vi "Ch_Apply.vi"(0 "Channels":T1(array[cluster]), 5 "Index":i32, 7 "Channel":T2={"Name"="CH000", "Value"=0.0, "High Limit"=100.0, "Low Limit"=0.0, "Save"=TRUE, "Graph"=FALSE, "Scale Min"=0.0, "Scale Max"=100.0, "Unit"="%"}, 9 "Apply All":bool, 11 "error in":errorcluster) -> (4 "Channels out":T1(array[cluster]), 15 "error out":errorcluster)   [LabVIEW 2026]
doc: "채널 설정 팝업 결과 반영: Apply All이면 상/하한·저장·그래프·스케일·단위를 128채널 모두에(이름/값 유지), 아니면 Index 채널만 교체."
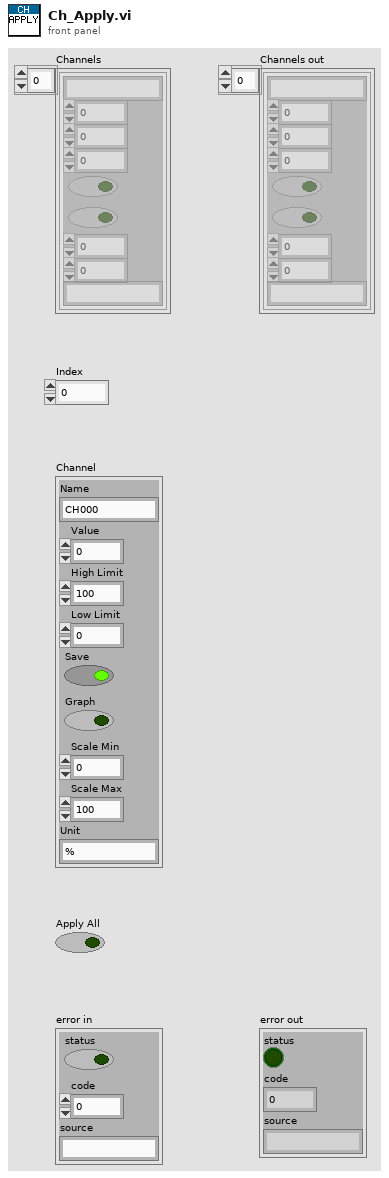
[diagram p1: front panel]
types:
  T1 = cluster{"Name":string, "Value":dbl, "High Limit":dbl, "Low Limit":dbl, "Save":bool, "Graph":bool, "Scale Min":dbl, "Scale Max":dbl, "Unit":string}[]
  T2 = cluster{"Name":string, "Value":dbl, "High Limit":dbl, "Low Limit":dbl, "Save":bool, "Graph":bool, "Scale Min":dbl, "Scale Max":dbl, "Unit":string}
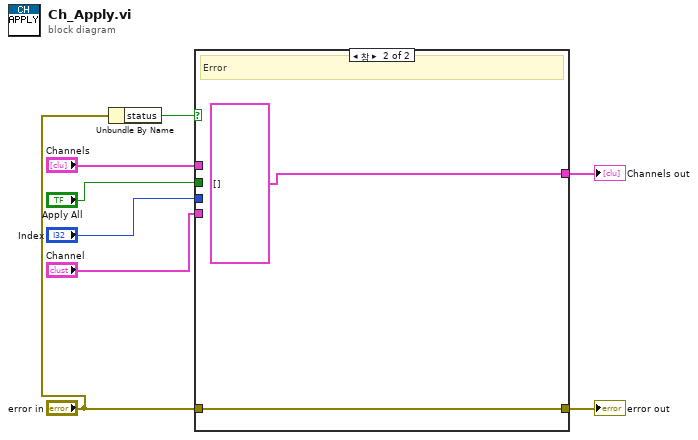
[diagram p0: block diagram]
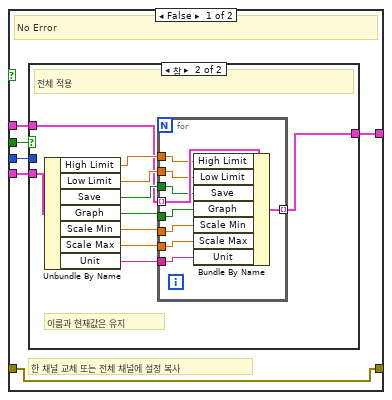
[diagram p2: hidden frame]
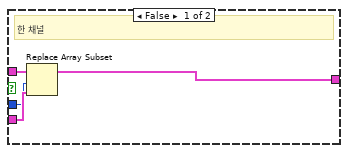
[diagram p3: hidden frame]
diagram:
  n1 = Unbundle By Name("error in") -> ("status"=w6:bool)
  n2 = case shown="참" w6 {
    tunnel: "Channels" -> [w9 _]
    tunnel: "Index" -> [w10 _]
    tunnel: "Channel" -> [w11 _]
    tunnel: "Apply All" -> [w12 _]
    tunnel: "error in" -> [w13 w38]
    tunnel: [w13 w38] -> w8
    tunnel: [w14 T1 []] -> w7
    frame False {
      # "한 채널 교체 또는 전체 채널에 설정 복사"
      # "No Error"
      n3 = case shown="참" w12 {
        tunnel: w9 -> [w15 w19]
        tunnel: w10 -> [w16 _]
        tunnel: w11 -> [w17 w20]
        tunnel: [w18 w28] -> w14
        frame False {
          # "한 채널"
          n4 = Replace Array Subset(array=w15, new element=w17, index=w16) -> (w18:T1)
        }
        frame True {
          # "이름과 현재값은 유지"
          # "전체 적용"
          n5 = Unbundle By Name(w20) -> ("High Limit"=w21:dbl, "Low Limit"=w22:dbl, "Save"=w23:bool, "Graph"=w24:bool, "Scale Min"=w25:dbl, "Scale Max"=w26:dbl, "Unit"=w27:string)
          n6 = for {
            tunnel: w19 -> [w36] mode=indexing
            tunnel: w21 -> [w29]
            tunnel: w22 -> [w30]
            tunnel: w23 -> [w31]
            tunnel: w24 -> [w32]
            tunnel: w25 -> [w33]
            tunnel: w26 -> [w34]
            tunnel: w27 -> [w35]
            tunnel: [w37] -> w28 mode=indexing
            n7 = Bundle By Name(cluster=w36, "High Limit"=w29, "Low Limit"=w30, "Save"=w31, "Graph"=w32, "Scale Min"=w33, "Scale Max"=w34, "Unit"=w35) -> (w37:T2)
          }
        }
      }
    }
    frame True {
      # "Error"
    }
  }
  "Channels out" <- w7
  "error out" <- w8
